vi "ReadName.vi"(8 "error in (no error)":errorcluster, 11 "Channel in":refnum<class "Channel.lvclass">) -> (0 "error out":errorcluster, 2 "Name":string, 3 "Channel out":refnum<class "Channel.lvclass">)   [LabVIEW 2021, in "Channel.lvlib" / "Channel.lvclass"]
uses:
  Channel.lvclass
  Configuration_class/Configuration.lvclass
  Channel.lvclass/Channel.ctl
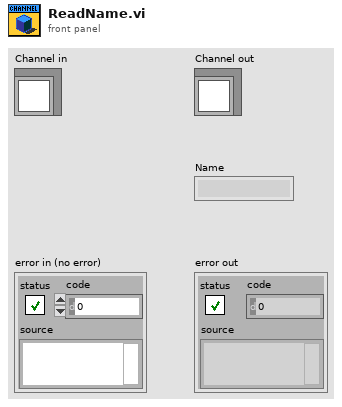
[diagram p1: front panel]
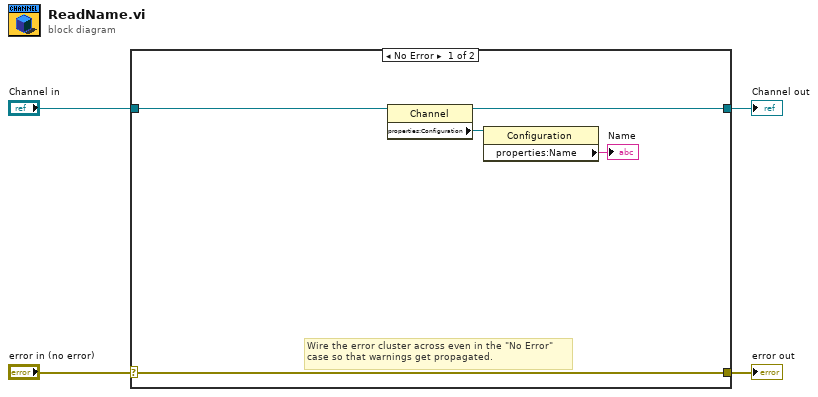
[diagram p0: block diagram]
diagram:
  n1 = case shown="No Error" "error in (no error)" {
    selector: "error in (no error)" -> [w8 w11]
    tunnel: [w8 w11] -> w3
    tunnel: [w7 w10] -> w1
    tunnel: "Channel in" -> [w9 w10]
    frame No Error {
      # "Wire the error cluster across even in the \"No Error\"\ncase so that warnings get propagated."
      n2 = property class="Channel"(reference=w9) -> (reference out=w7:refnum<class "Channel.lvclass">, "properties:Configuration"=w6:refnum<class "Configuration.lvclass">)  [unwired: 1 in, 1 out]
      n3 = property class="Configuration"(reference=w6) -> ("properties:Name"=→"Name":string)  [unwired: 1 in, 2 out]
    }
    frame Error {
    }
  }
  "error out" <- w3
  "Channel out" <- w1
